vi "PicoScope4000aGetValuesOverlappedBulk.vi"(5 "Segment Range":T1 {"toSegmentIndex" format="%.4p"; "fromSegmentIndex" format="%.4p"}, 7 "Buffer and Transfer Settings":T2 {"Down-Sample Mode" items=["None", "Aggregate", "Decimate", "Average"]; "Down Sample Ratio" step=1; "Samples" format="%_6p"}, 8 "error in (no error)":errorcluster, 11 "handle in":i16) -> (0 "error out":errorcluster, 3 "handle out":i16, 4 "Pointer to Overflow":u64[](array[numeric]), 6 "noOfSamples":u64)   [LabVIEW 2009]
doc: "Calls GetValuesOverlappedBulk"
uses:
  Program Files/Pico Technology/SDK/lib/ps4000a.dll
  shared/Buffer and Transfer Settings.ctl
  shared/Segment Range.ctl
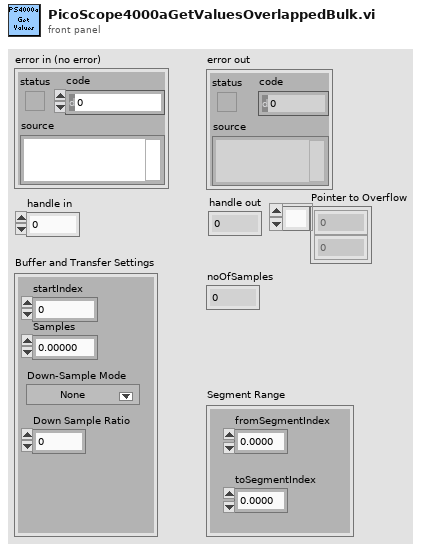
[diagram p1: front panel]
types:
  T1 = typedef "Segment Range.ctl" = cluster{"fromSegmentIndex":u64, "toSegmentIndex":u64}
  T2 = typedef "Buffer and Transfer Settings.ctl" = cluster{"startIndex":u64, "Samples":u64, "Down Sample Ratio":u64, "Down-Sample Mode":u32}
  T3 = cluster{"status":bool, "code":u32, "source":string}
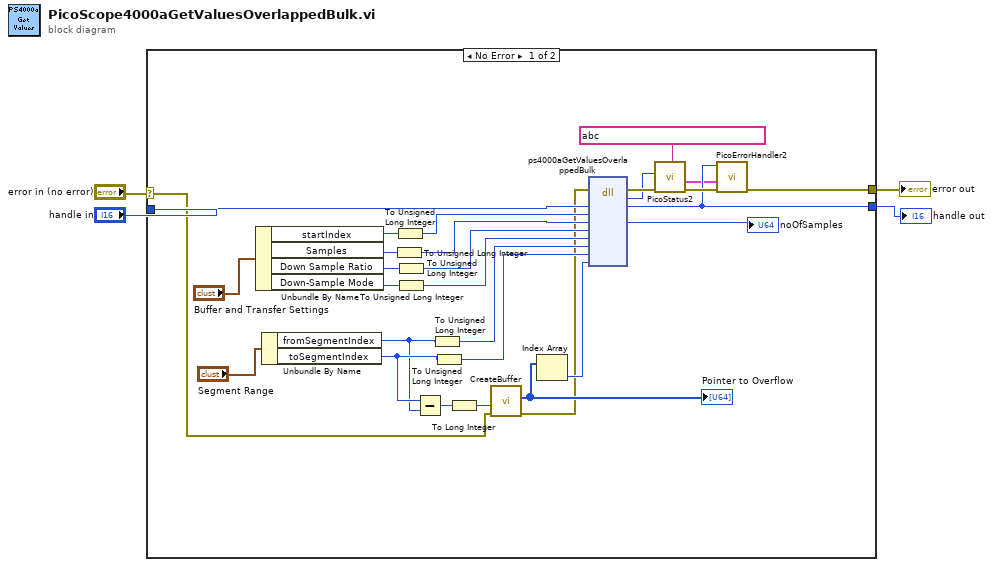
[diagram p0: block diagram]
diagram:
  n1 = case shown="No Error" "error in (no error)" {
    selector: "error in (no error)" -> [w6 w34]
    tunnel: "handle in" -> [w24 w35]
    tunnel: [w27 w35] -> w4
    tunnel: [w30 w34] -> w3
    frame #0 {
      n2 = Unbundle By Name("Buffer and Transfer Settings") -> ("startIndex"=w19:u64, "Samples"=w17:u64, "Down Sample Ratio"=w16:u64, "Down-Sample Mode"=w15:u32)
      n3 = Unbundle By Name("Segment Range") -> ("fromSegmentIndex"=w22:u64, "toSegmentIndex"=w23:u64)
      n4 = To Unsigned Long Integer(number=w17) -> (unsigned 32bit integer=w14:u32)
      n5 = To Unsigned Long Integer(number=w19) -> (unsigned 32bit integer=w18:u32)
      n6 = To Unsigned Long Integer(number=w16) -> (unsigned 32bit integer=w13:u32)
      n7 = To Unsigned Long Integer(number=w15) -> (unsigned 32bit integer=w12:u32)
      n8 = Subtract(x=w23, y=w22) -> (x-y=w25:u64)
      n9 = To Unsigned Long Integer(number=w22) -> (unsigned 32bit integer=w21:u32)
      n10 = To Unsigned Long Integer(number=w23) -> (unsigned 32bit integer=w20:u32)
      n11 = To Long Integer(number=w25) -> (32bit integer=w9:i32)
      n12 = call "CreateBuffer.vi"("error in (no error)"=w6, "Buffer size"=w9) -> ("error out"=w7:errorcluster, "Pointer and BufferSize"=w10:u64[])  [unwired: 8 in]
      "Pointer to Overflow" <- w10
      n13 = Index Array(array=w10) -> (element=w8:u64)  [unwired: 1 in]
      n14 = dll-call lib="/Program Files/Pico Technology/SDK/lib/ps4000a.dll" fn="ps4000aGetValuesOverlappedBulk" ("ps3000.dll:_ps3000_open_unit@0")(error in=w7, "handle"=w24, "startIndex"=w18, "noOfSamples"=w14, "downSampleRatio"=w13, "downSampleRatioMode"=w12, "fromSegmentIndex"=w21, "toSegmentIndex"=w20, "overflow"=w8) -> (error out=w28:errorcluster, "PICO_STATUS"=w26:u32, "handle"=w27:i16, "noOfSamples"=→"noOfSamples":u32)  [unwired: 8 in, 1 out]
      n15 = call "PicoStatus2.vi"("PICO source"=string ? ("source"), "Error in"=w28, "PICO STATUS"=w26) -> ("error out"=w33:errorcluster, "PICO_STATUS out"=w5:T3)  [unwired: 5 in]
      n16 = call "PicoErrorHandler2.vi"("error in (no error)"=w33, "PICO_STATUS in"=w5, "handle In"=w27) -> ("error out"=w30:errorcluster)  [unwired: 8 in]
    }
    frame #1 {
    }
  }
  "error out" <- w3
  "handle out" <- w4
